vi "ble_parse_scan_response.vi"(11 "Scan Response Data":u8[](array[numeric]) format="%02x") -> (3 "Array Scan Response":string[](array[string]))   [LabVIEW 2013]
uses:
  type_def/advertising_package_type.ctl
  type_def/address_type.ctl
panel:
  out "Friendly Name":string
  out "RSSI string":string
  out "Addvertiser Address Type":string
  in  "Address Type":T1 items=["Public", "Random"]
  out "MAC string OUT colon":string
  out "Advertising Package Type String":string
  in  "Advertising Package Type":T2 items=["Connectable Advertisement packet"=0, "Non Connectable Advertisement packet"=2, "Scan response packet"=4, "Discoverable advertisement packet"=6]
  out "RSSI (dBm)":i8
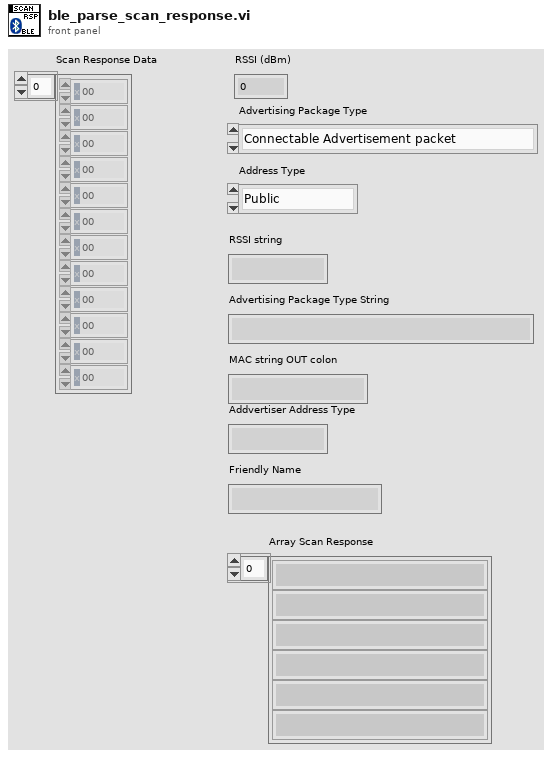
[diagram p1: front panel]
types:
  T1 = typedef "address_type.ctl" = u8
  T2 = typedef "advertising_package_type.ctl" = u8
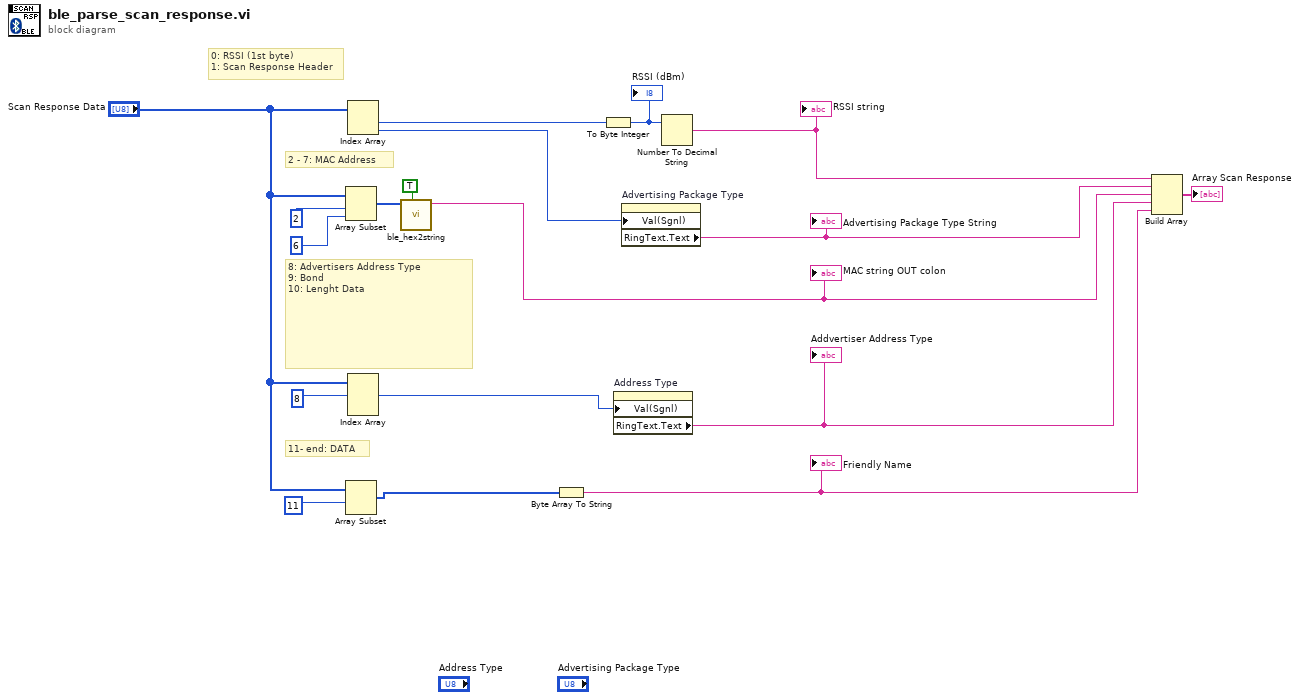
[diagram p0: block diagram]
diagram:
  # "11- end: DATA"
  # "8: Advertisers Address Type\n9: Bond\n10: Lenght Data"
  # "2 - 7: MAC Address"
  # "0: RSSI (1st byte)\n1: Scan Response Header"
  n1 = Array Subset(array="Scan Response Data", index=2, length=6) -> (w6:u8[])
  n2 = Array Subset(array="Scan Response Data", index=11 ("length")) -> (w1:u8[])  [unwired: 1 in]
  n3 = Index Array(array="Scan Response Data") -> (element #1=w18:u8, element #2=w12:u8)  [unwired: 2 in]
  n4 = Index Array(array="Scan Response Data", index #1=8 ("length")) -> (element #1=w11:u8)  [unwired: 2 in, 2 out]
  n5 = call "ble_hex2string.vi"("colon?(false)"=TRUE, "Byte Array IN (index0 LS byte)"=w6) -> ("HEX string OUT"=w5:string)  [unwired: 9 in]
  "MAC string OUT colon" <- w5
  n6 = Byte Array To String(unsigned byte array=w1) -> (string=w2:string)
  "Friendly Name" <- w2
  n7 = To Byte Integer(number=w18) -> (8bit integer=w15:i8)
  "RSSI (dBm)" <- w15
  n8 = property on="Address Type" class="Ring (strict)"("Val(Sgnl)"=w11) -> ("RingText.Text"=w8:string)  [unwired: 2 in, 2 out]
  "Addvertiser Address Type" <- w8
  n9 = property on="Advertising Package Type" class="Ring (strict)"("Val(Sgnl)"=w12) -> ("RingText.Text"=w9:string)  [unwired: 2 in, 2 out]
  "Advertising Package Type String" <- w9
  n10 = Number To Decimal String(number=w15) -> (decimal integer string=w10:string)  [unwired: 1 in]
  "RSSI string" <- w10
  n11 = Build Array(w10, w9, w5, w8, w2) -> (→"Array Scan Response":string[])
